vi "Folder Reuse Warning.vi"(8 "error in":errorcluster, 10 "folder names":string[](array[string]), 11 "project ref":refnum<vi>) -> (0 "error out":errorcluster, 3 "proceed?":bool)   [LabVIEW 2021, in "MeasurementClient Editor.lvlib"]
uses:
  MeasurementClient Editor.lvlib
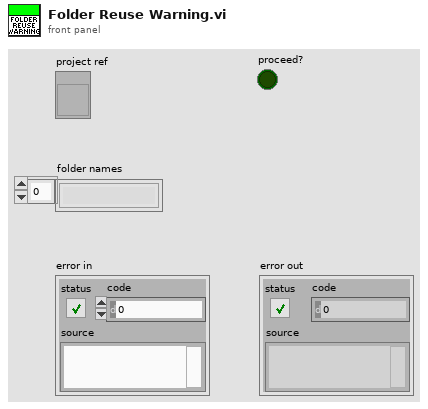
[diagram p1: front panel]
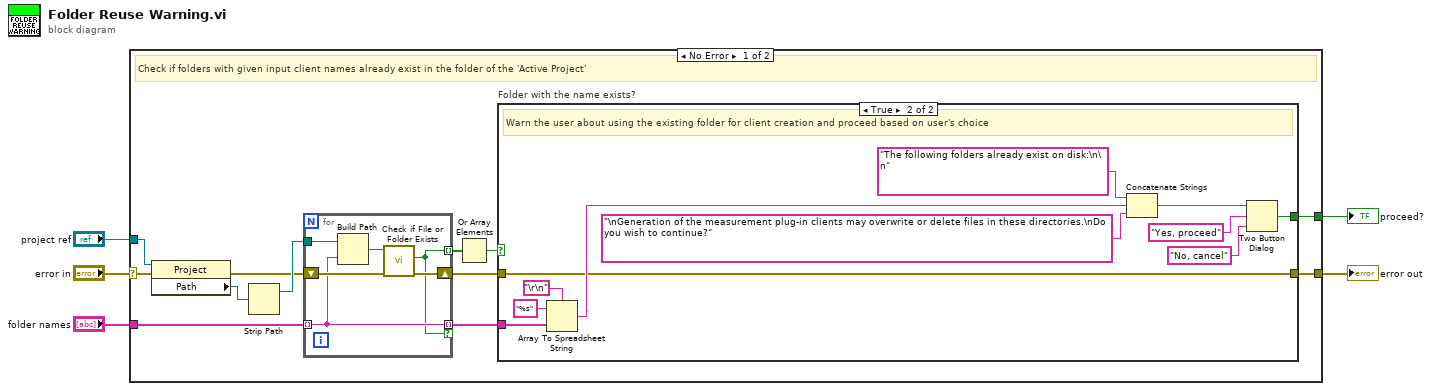
[diagram p0: block diagram]
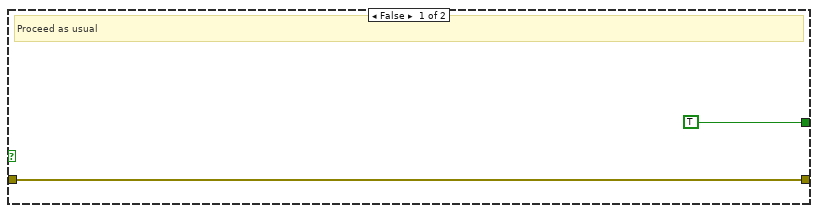
[diagram p2: hidden frame]
diagram:
  n1 = case shown="No Error" "error in" {
    selector: "error in" -> [w17 w37]
    tunnel: [w13 w37] -> w2
    tunnel: "folder names" -> [w12 _]
    tunnel: "project ref" -> [w6 _]
    tunnel: [w9 _] -> w1
    frame No Error {
      # "Check if folders with given input client names already exist in the folder of the 'Active Project'"
      n2 = property class="Project"(reference=w6, error in=w17) -> (error out=w8:errorcluster, "Path"=w16:path)  [unwired: 1 out]
      n3 = Strip Path(path=w16) -> (stripped path=w15:path)  [unwired: 1 out]
      n4 = for {
        tunnel: w15 -> [w36]
        tunnel: w12 -> [w32] mode=indexing
        tunnel: [w31] -> w14 mode=indexing
        tunnel: [w32] -> w11 mode=indexing if=w31
        shift-right: [w33] -> w7
        shift-left: w8 -> [w34]
        n5 = Build Path(base path=w36, name or relative path=w32) -> (appended path=w35:path)
        n6 = call <vilib>:"Check if File or Folder Exists.vi"("error in (no error)"=w34, "path"=w35) -> ("error out"=w33:errorcluster, "file or folder exists?"=w31:bool)  [unwired: 7 in, 1 out]
      }
      n7 = Or Array Elements(Boolean array=w14) -> (logical OR=w10:bool)
      n8 = case "Folder with the name exists?" shown="True" w10 {
        tunnel: [w19 w25] -> w13
        tunnel: w11 -> [_ w30]
        tunnel: [TRUE ("T button?") w27] -> w9
        tunnel: w7 -> [w19 w25]
        frame False {
          # "Proceed as usual"
        }
        frame True {
          # "Warn the user about using the existing folder for client creation and proceed based on user's choice"
          n9 = Array To Spreadsheet String(delimiter (Tab)="\r\n", array=w30, 3:"%s" ("format string")) -> (spreadsheet string=w28:string)
          n10 = Concatenate Strings("The following folders already exist on disk:\n\n" ("string"), w28, "\nGeneration of the measurement plug-in clients may overwrite or delete files in these directories.\nDo you wish to continue?" ("string")) -> (w22:string)
          n11 = Two Button Dialog(message=w22, 1:"No, cancel" ("F button name (\"Cancel\")"), 2:"Yes, proceed" ("T button name (\"OK\")")) -> (T button?=w27:bool)
        }
      }
    }
    frame Error {
      # "Pass"
    }
  }
  "error out" <- w2
  "proceed?" <- w1
